vi "Get Config File.vi"(8 "error in (no error)":errorcluster) -> (0 "error out":errorcluster, 3 "Config File":path)   [LabVIEW 2021, in "Channel.lvlib"]
uses:
  Channel.lvlib
  Private/G_Paths.vi
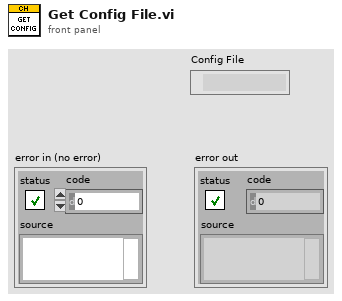
[diagram p1: front panel]
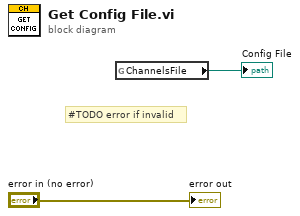
[diagram p0: block diagram]
diagram:
  # "#TODO error if invalid"
  n1 = global read "G_Paths.vi" "ChannelsFile"() -> (→"Config File":path)
  "error out" <- "error in (no error)"
